vi "PicoScope4000aRunBlock.vi"(7 "Acquisition Settings":T1={"preTriggerSamples"=0, "postTriggerSamples"=1000, "timebase"=2} {"postTriggerSamples" format="%_6p"; "preTriggerSamples" format="%_6p"}, 8 "error in (no error)":errorcluster, 11 "handle in":i16) -> (0 "error out":errorcluster, 3 "handle out":i16, 4 "timeIndisposedMs":dbl, 6 "Total Requested Samples":u64)   [LabVIEW 2010]
doc: "Calls RunBlock"
uses:
  ps4000a.dll
  shared/Acquisition Settings.ctl
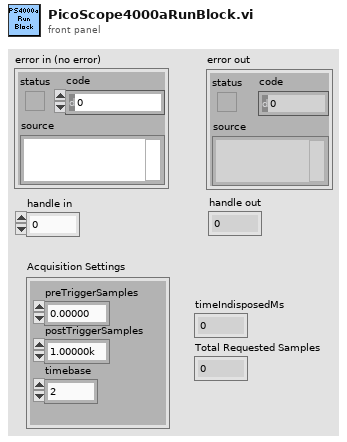
[diagram p1: front panel]
types:
  T1 = typedef "Acquisition Settings.ctl" = cluster{"preTriggerSamples":u64, "postTriggerSamples":u64, "timebase":u32}
  T2 = cluster{"status":bool, "code":u32, "source":string}
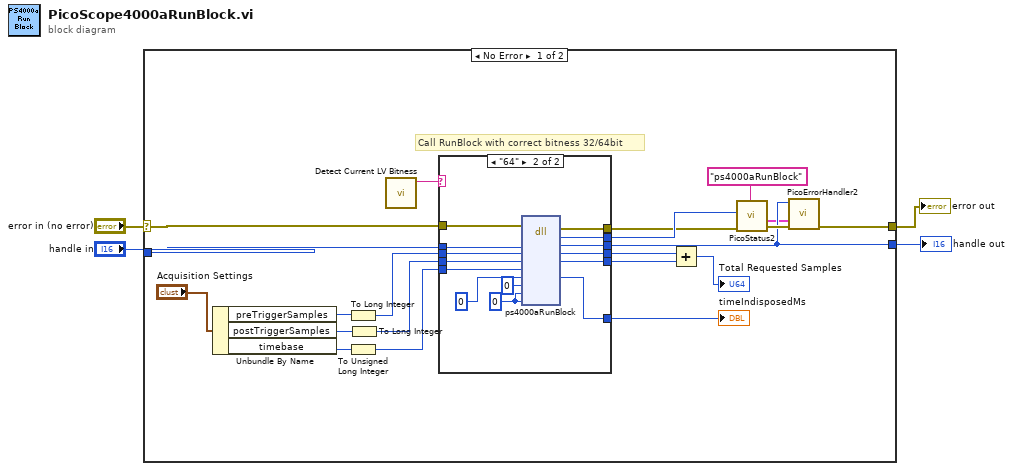
[diagram p0: block diagram]
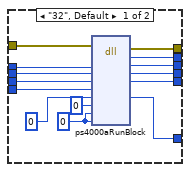
[diagram p2: hidden frame]
diagram:
  n1 = case shown="No Error" "error in (no error)" {
    selector: "error in (no error)" -> [w19 w55]
    tunnel: [w15 w55] -> w2
    tunnel: "handle in" -> [w18 w54]
    tunnel: [w14 w54] -> w3
    frame No Error {
      # "Call RunBlock with correct bitness 32/64bit"
      n2 = Unbundle By Name("Acquisition Settings") -> ("preTriggerSamples"=w11:u64, "postTriggerSamples"=w9:u64, "timebase"=w10:u32)
      n3 = To Long Integer(number=w11) -> (32bit integer=w8:i32)
      n4 = To Unsigned Long Integer(number=w10) -> (unsigned 32bit integer=w6:u32)
      n5 = To Long Integer(number=w9) -> (32bit integer=w7:i32)
      n6 = call "Detect Current LV Bitness.vi"() -> ("bitness"=w16:string)  [unwired: 11 in]
      n7 = case shown="\"64\"" w16 {
        tunnel: [w39 w53] -> w25
        tunnel: [w38 w52] -> w24
        tunnel: [w37 w51] -> w22
        tunnel: [w36 w50] -> w21
        tunnel: w19 -> [w35 w49]
        tunnel: w18 -> [w34 w48]
        tunnel: w8 -> [w32 w46]
        tunnel: w7 -> [w31 w45]
        tunnel: w6 -> [w30 w44]
        tunnel: [w29 w43] -> w14
        tunnel: [w26 w41] -> w13
        frame "32", Default {
          w28 = u32 0 ("pParameter")
          n8 = dll-call lib="ps4000a.dll" fn="ps4000aRunBlock" ("ps3000.dll:_ps3000_open_unit@0")(error in=w35, "handle"=w34, "noOfPreTriggerSamples"=w32, "noOfPostTriggerSamples"=w31, "timebase"=w30, "timeIndisposedMs"=0 ("pParameter"), "segmentIndex"=u32 0, "lpReady"=w28, "pParameter"=w28) -> (error out=w36:errorcluster, "PICO_STATUS"=w37:u32, "handle"=w29:i16, "noOfPreTriggerSamples"=w39:i32, "noOfPostTriggerSamples"=w38:i32, "timeIndisposedMs"=w26:i32)  [unwired: 6 in, 1 out]
        }
        frame "64" {
          w42 = u64 0 ("pParameter")
          n9 = dll-call lib="ps4000a.dll" fn="ps4000aRunBlock" ("ps3000.dll:_ps3000_open_unit@0")(error in=w49, "handle"=w48, "noOfPreTriggerSamples"=w46, "noOfPostTriggerSamples"=w45, "timebase"=w44, "timeIndisposedMs"=0 ("pParameter"), "segmentIndex"=u32 0, "lpReady"=w42, "pParameter"=w42) -> (error out=w50:errorcluster, "PICO_STATUS"=w51:u32, "handle"=w43:i16, "noOfPreTriggerSamples"=w53:i32, "noOfPostTriggerSamples"=w52:i32, "timeIndisposedMs"=w41:i32)  [unwired: 6 in, 1 out]
        }
      }
      "timeIndisposedMs" <- w13
      n10 = Add(x=w25, y=w24) -> (x+y=→"Total Requested Samples":i32)
      n11 = call "PicoStatus2.vi"("PICO source"="ps4000aRunBlock" ("source"), "Error in"=w21, "PICO STATUS"=w22) -> ("error out"=w17:errorcluster, "PICO_STATUS out"=w5:T2)  [unwired: 5 in]
      n12 = call "PicoErrorHandler2.vi"("error in (no error)"=w17, "PICO_STATUS in"=w5, "handle In"=w14) -> ("error out"=w15:errorcluster)  [unwired: 8 in]
    }
    frame Error {
    }
  }
  "error out" <- w2
  "handle out" <- w3
